vi "DPI Configuration.vi"(11 "DPE Project File Path":string) -> (3 "DPI Instrument Name":refnum<k15>)   [LabVIEW 2025, in "Digital Pattern Sequencer.lvclass"]
uses:
  Digital Pattern Sequencer.lvclass
  Digital Pattern Sequencer.lvclass/Digital Pattern Sequencer.ctl
  <instrlib>/niDigital/niDigital.llb/niDigital Load Specifications Levels and Timing (Single).vi
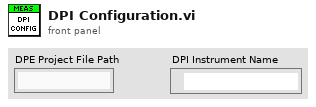
[diagram p1: front panel]
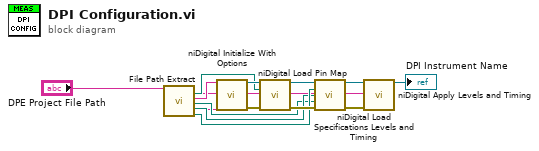
[diagram p0: block diagram]
diagram:
  n1 = call "File Path Extract.vi"("DPE Project File Path"="DPE Project File Path") -> ("Timing path name"=w2:string, "Level path name"=w3:string, ".pinmap file path"=w10:path, "DPI Instrument Name"=w14:string, ".digitiming file path"=w4:path, ".digilevels file path"=w5:path, ".spec file path"=w6:path)  [unwired: 10 in, 2 out]
  n2 = call <instrlib>:"niDigital Initialize With Options.vi"("resource name"=w14) -> ("instrument handle"=w11:refnum<k15>, "error out"=w9:errorcluster)  [unwired: 13 in]
  n3 = call <instrlib>:"niDigital Load Pin Map.vi"("instrument handle"=w11, "pin map file"=w10, "error in"=w9) -> ("instrument handle out"=w12:refnum<k15>, "error out"=w8:errorcluster)  [unwired: 11 in]
  n4 = call-poly <instrlib>:"niDigital Load Specifications Levels and Timing.vi"("instrument handle"=w12, "specifications file path"=w6, "levels file path"=w5, "timing file path"=w4, "error in"=w8) -> ("instrument handle out"=w13:refnum<k15>, "error out"=w7:errorcluster)  [unwired: 9 in]
  n5 = call <instrlib>:"niDigital Apply Levels and Timing.vi"("instrument handle"=w13, "levels sheet"=w3, "timing sheet"=w2, "error in"=w7) -> ("instrument handle out"=→"DPI Instrument Name":refnum<k15>)  [unwired: 10 in, 1 out]
